vi "[ce] MsgBox - About CalcExpress.vi"(7 "custom title":string, 8 "error in":errorcluster, 9 "message after...":string, 10 "complete info (T)":bool=TRUE, 11 "message before...":string) -> (0 "error out":errorcluster)   [LabVIEW 2021]
doc: "Opens a dialog box displaying information about the CalcExpress Toolkit.\n\n::: CalcExpress Toolkit :::\nCopyright (c) 2000-2026 Konstantin Shifershteyn. All rights reserved."
uses:
  <vilib>/Platform/browser.llb/Open URL in Default Browser (string).vi
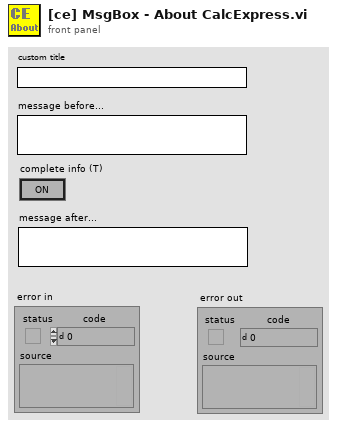
[diagram p1: front panel]
types:
  T1 = cluster{"Left Button Key Shortcut":cluster{"Control":bool, "Shift":bool, "Key":string}, "Center Button Key Shortcut":cluster{"Control":bool, "Shift":bool, "Key":string}, "Right Button Key Shortcut":cluster{"Control":bool, "Shift":bool, "Key":string}}
  T2 = cluster{"File Description":string, "Company Name":string, "File Version":string, "Internal Name":string, "Original Filename":string, "Product Name":string, "Product Version":string, "Copyright":string, "Trademarks":string, "Comments":string, "Build date":string, "Build version":string}
  T3 = enum32{"invalid app kind", "Development System", "Run Time System", "Student Edition", "Embedded LabVIEW", "Evaluation", "Custom"}
  T4 = enum16{"Left Button", "Center Button", "Right Button", "Window Close"}
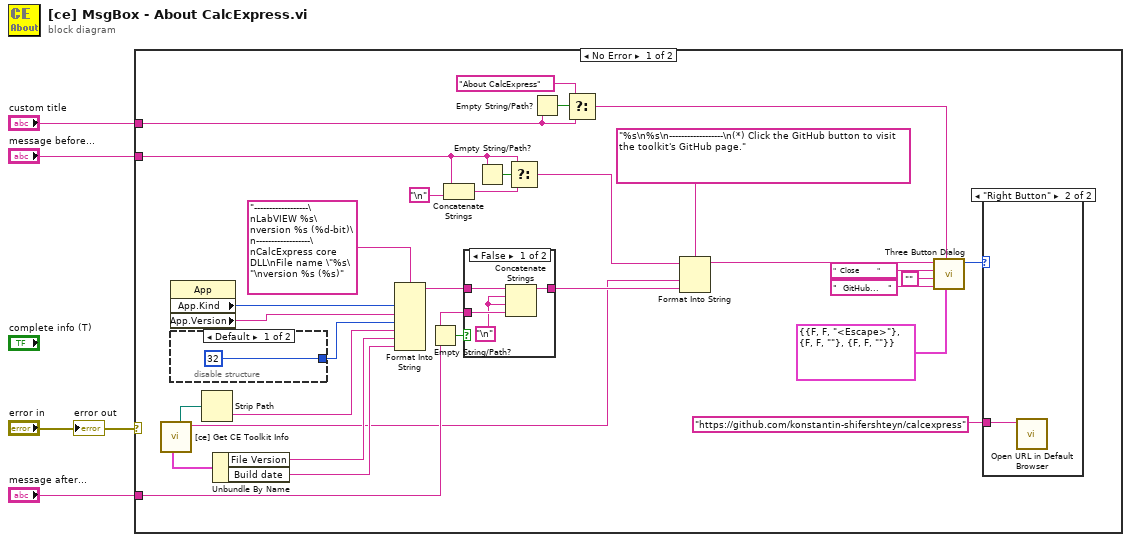
[diagram p0: block diagram]
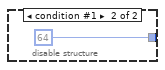
[diagram p4: hidden frame]
diagram:
  n1 = case shown="No Error" "error in" {
    tunnel: "custom title" -> [w35 _]
    tunnel: "message before..." -> [w9 _]
    tunnel: "message after..." -> [w29 _]
    frame No Error {
      n2 = call "[ce] Get CE Toolkit Info.vi"() -> ("LicenseInfo"=w13:string, "CE Engine Path"=w25:path, "CE DLL Info"=w26:T2)  [unwired: 4 in, 5 out]
      n3 = property class="App"() -> ("App.Kind"=w32:T3, "App.Version"=w33:string)  [unwired: 2 in, 2 out]
      n4 = disable-structure shown="Default" {
        disable-tunnel: [32 64] -> w34
        frame condition #0 (active) {
        }
        frame condition #1 {
        }
      }
      n5 = Strip Path(path=w25) -> (name=w24:string)  [unwired: 1 out]
      n6 = Unbundle By Name(w26) -> ("File Version"=w23:string, "Build date"=w22:string)
      n7 = Format Into String(format string="------------------\nLabVIEW %s\nversion %s (%d-bit)\n------------------\nCalcExpress core DLL\nFile name \"%s\"\nversion %s (%s)", w32, w33, w34, w24, w23, w22) -> (resulting string=w30:string)  [unwired: 2 in, 1 out]
      n8 = Empty String/Path?(string/path=w29) -> (empty?=w28:bool)
      n9 = Concatenate Strings(w9, "\n") -> (w12:string)
      n10 = case shown="False" w28 {
        tunnel: w30 -> [w40 w41]
        tunnel: w29 -> [w39 _]
        tunnel: [w38 w41] -> w27
        frame False {
          w37 = "\n"
          n11 = Concatenate Strings(w40, w37, w37, w39) -> (w38:string)
        }
        frame True {
        }
      }
      n12 = Empty String/Path?(string/path=w9) -> (empty?=w8:bool)
      n13 = Select(t=w9, s=w8, f=w12) -> (s? t:f=w10:string)
      n14 = Empty String/Path?(string/path=w35) -> (empty?=w21:bool)
      n15 = Select(t="About CalcExpress", s=w21, f=w35) -> (s? t:f=w20:string)
      n16 = Format Into String(format string="%s\n%s\n------------------\n(*) Click the GitHub button to visit the toolkit's GitHub page.", initial string=w10, w13, w27) -> (resulting string=w17:string)  [unwired: 1 in, 1 out]
      n17 = call <vilib>:"Three Button Dialog.vi"("Keyboard Shortcuts (Left is <Enter>)"=T1 {"Left Button Key Shortcut"={"Control"=FALSE, "Shift"=FALSE, "Key"="<Escape>"}, "Center Button Key Shortcut"={"Control"=FALSE, "Shift"=FALSE, "Key"=""}, "Right Button Key Shortcut"={"Control"=FALSE, "Shift"=FALSE, "Key"=""}}, "Window Title (\"\")"=w20, "Right Button Text (\"Cancel\")"="  GitHub...   ", "Center Button Text (\"No\")"="", "Left Button Text (\"Yes\")"="  Close         " ("Left Button Text (\"Yes\")"), "message"=w17) -> ("Which Button?"=w6:T4)  [unwired: 5 in]
      n18 = case shown="\"Right Button\"" w6 {
        tunnel: "https://github.com/konstantin-shifershteyn/calcexpress" -> [_ w36]
        frame Default {
        }
        frame "Right Button" {
          n19 = call-poly <vilib>:"Open URL in Default Browser.vi"("URL"=w36) -> ()  [unwired: 5 in, 2 out]
        }
      }
    }
    frame Error {
    }
  }
  "error out" <- "error in"
